vi "CP for Time Vi_MS.vi"(8 "CP A Tag":string[](array[string]), 11 "CP Profile Table for All Seql":string[][](table)) -> (3 "CPIDXZ":T1)   [LabVIEW 2018]
panel:
  out "M_MxRight_No":string[](array[string])
  out "M_RRead_Seq":string[](array[string])
  out "Mx Right No":string[](array[string])
  out "Mx Right Read Seq":string[](array[string])
  out "Assinged Sequence":string[](array[string])
  out "Direction":string[](array[string])
  out "MS_IDX":string[](array[string])
  out "Mx Intensity level [pA]":string[](array[string])
  out "BLX Level [pA]":string[](array[string])
  out "Signal Intensity [pA]":string[](array[string])
  out "S/N ratio":string[](array[string])
  out "S#_IDX":string[](array[string])
  out "L#_IDX":string[](array[string])
  out "AS IDX":string[](array[string])
  out "CP T IDX End [n]":string[](array[string])
  out "CP T IDX Start [n]":string[](array[string])
  out "サイズ":i32
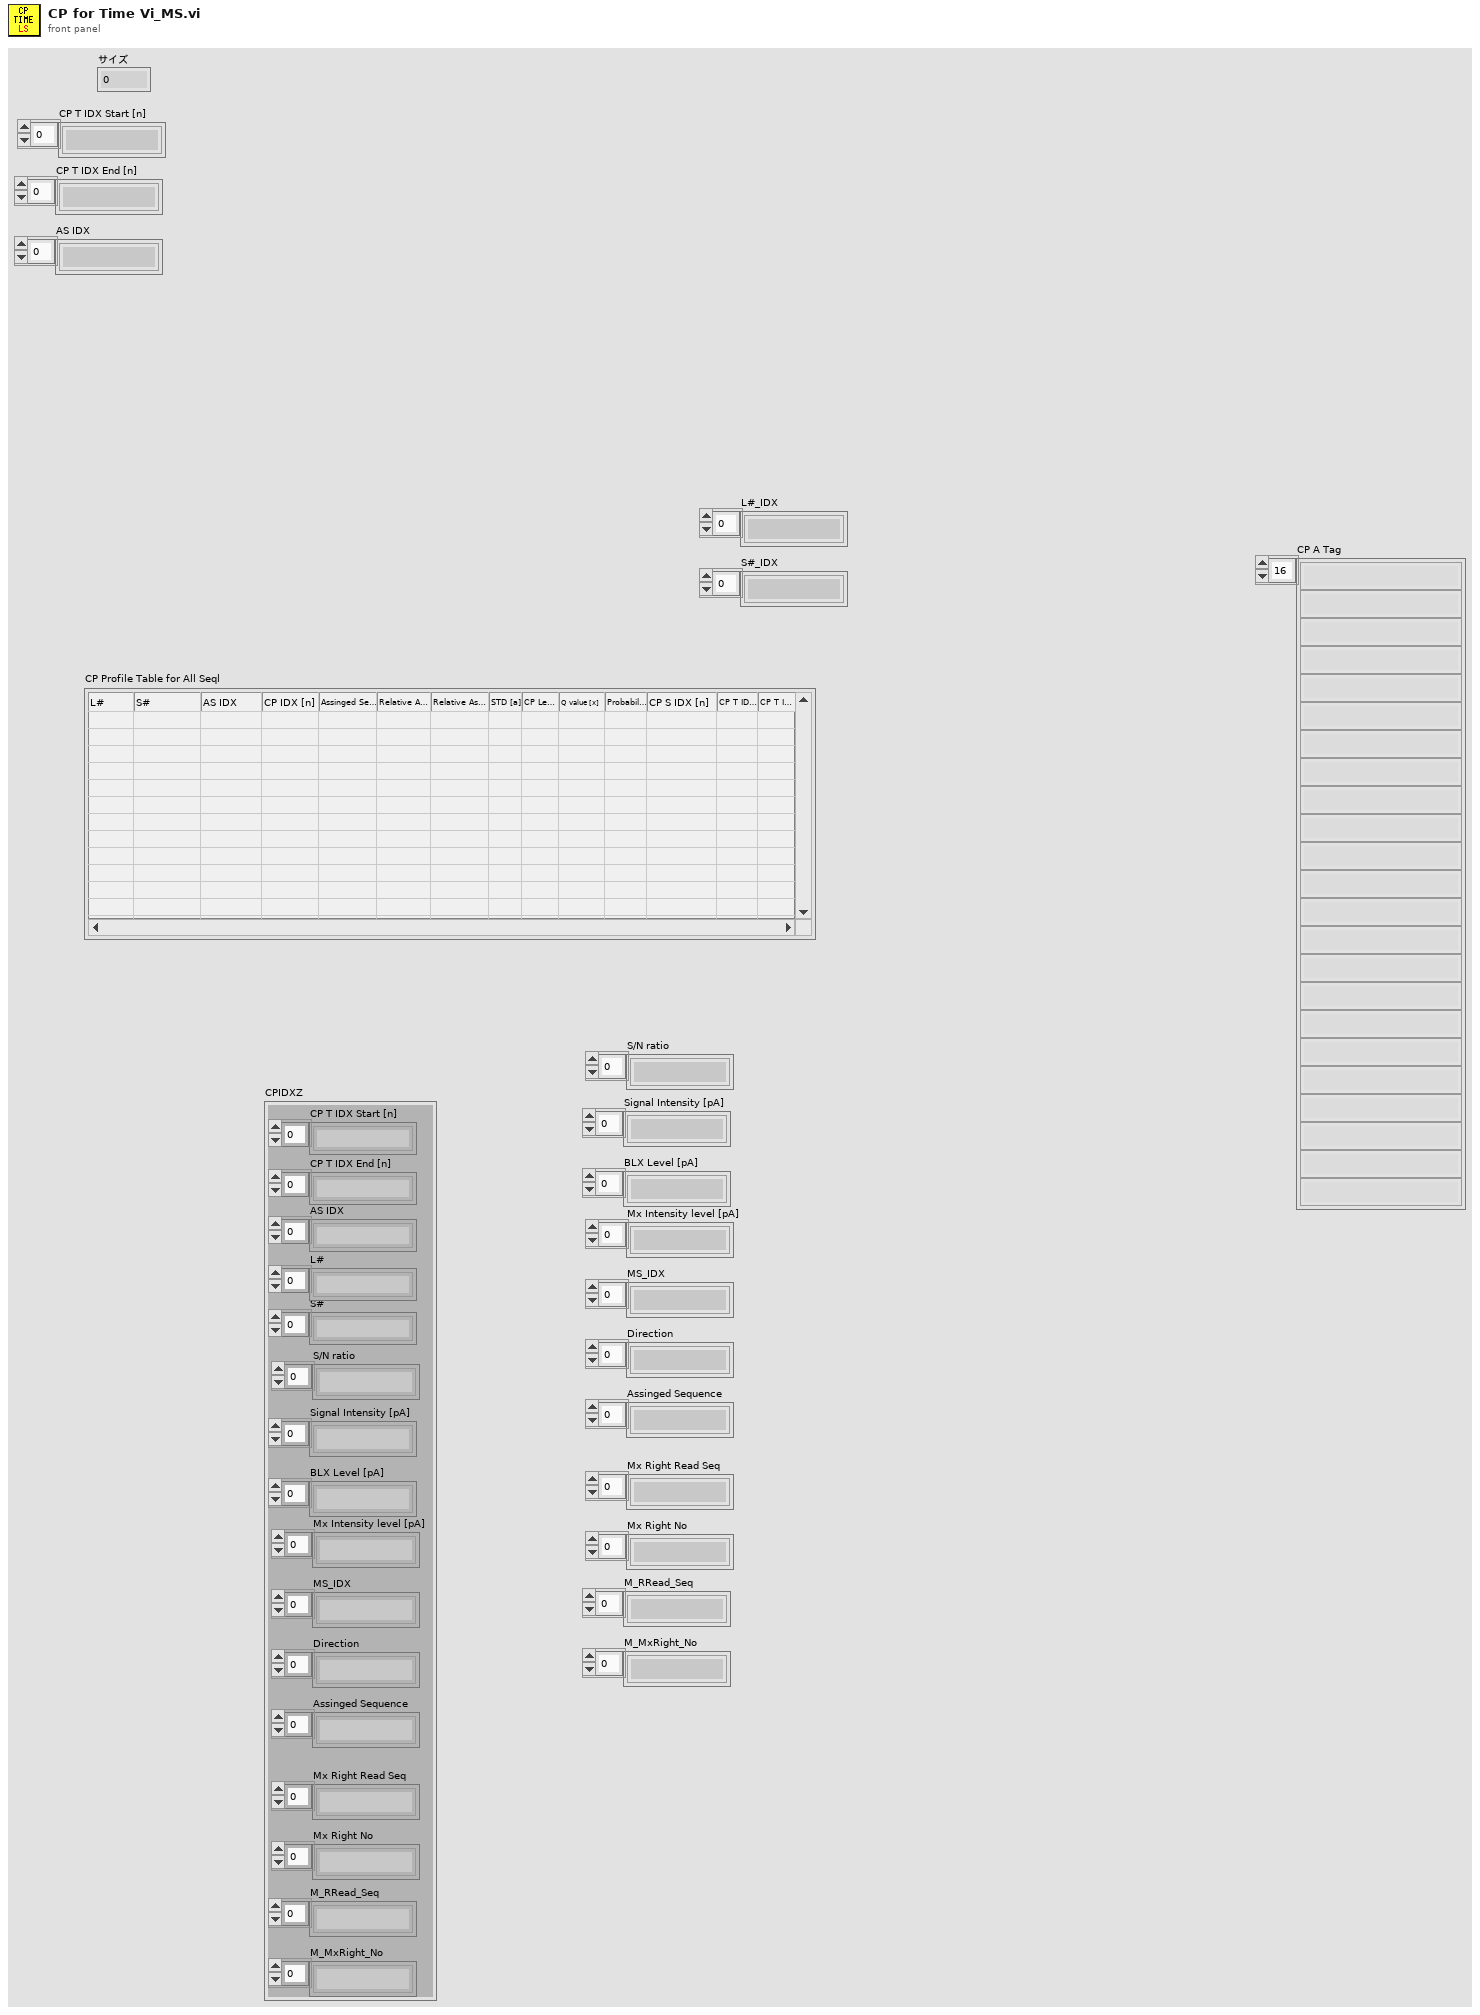
[diagram p1: front panel]
types:
  T1 = cluster{"CP T IDX Start [n]":string[], "CP T IDX End [n]":string[], "AS IDX":string[], "L#":string[], "S#":string[], "S/N ratio":string[], "Signal Intensity [pA]":string[], "BLX Level [pA]":string[], "Mx Intensity level [pA]":string[], "MS_IDX":string[], "Direction":string[], "Assinged Sequence":string[], "Mx Right Read Seq":string[], "Mx Right No":string[], "M_RRead_Seq":string[], "M_MxRight_No":string[]}
  T2 = cluster{string[], string[], string[], string[], string[], string[], string[], string[], string[], string[], string[], string[], string[], string[], string[], string[]}
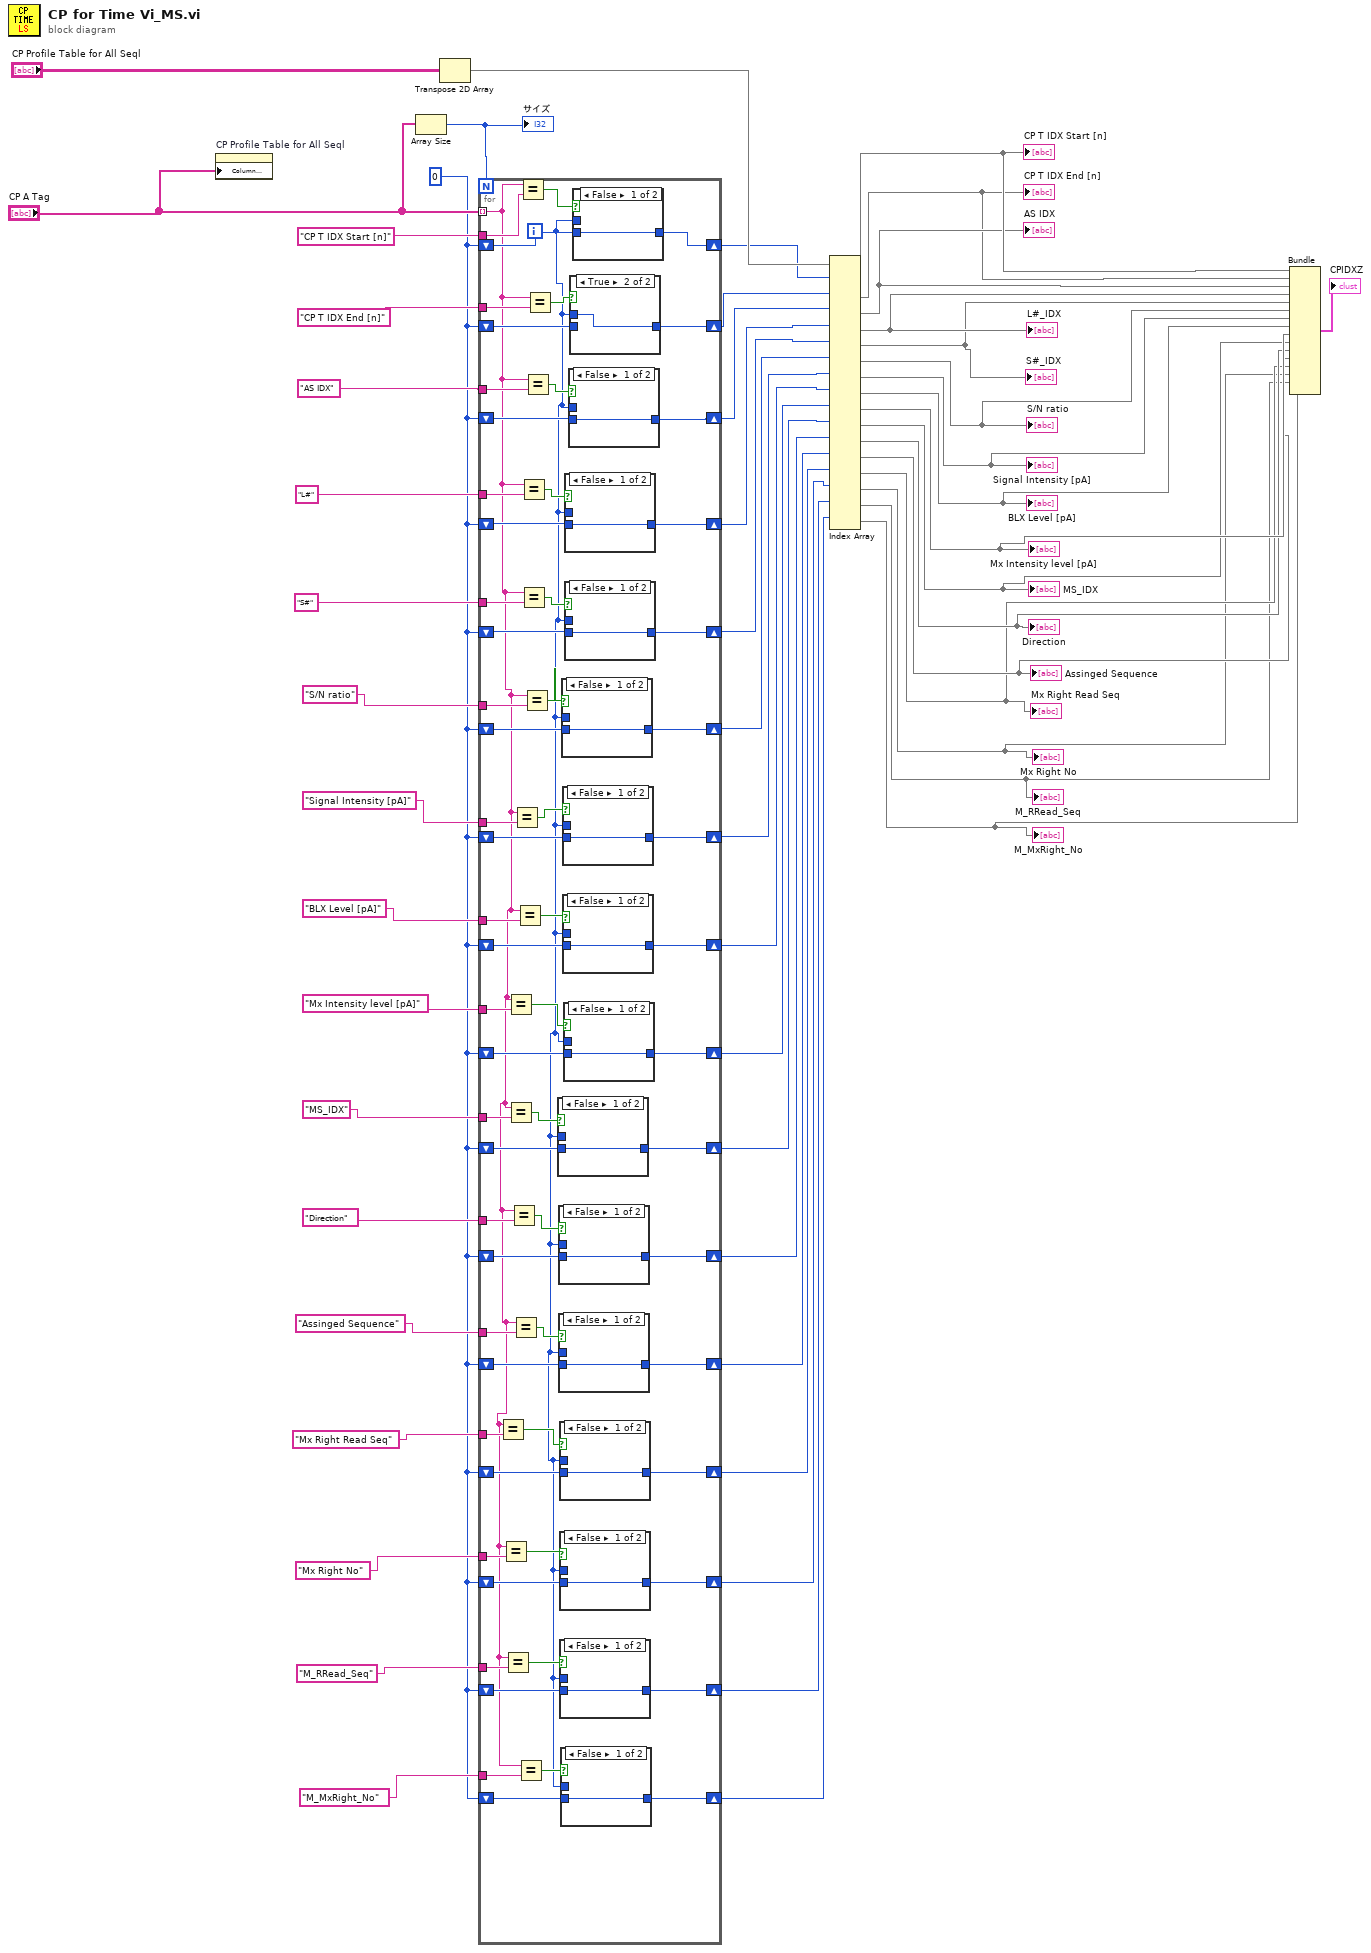
[diagram p0: block diagram]
diagram:
  w24 = 0
  n1 = property on="CP Profile Table for All Seql" class="Tbl (strict)"("Column Headers[]"="CP A Tag") -> ()  [unwired: 2 in, 2 out]
  n2 = Array Size(array="CP A Tag") -> (size(s)=w54:i32)
  "サイズ" <- w54
  n3 = Transpose 2D Array(2D array="CP Profile Table for All Seql") -> (transposed array=w53:string[][])
  n4 = for {
    N: w54 -> [_]
    tunnel: "CP A Tag" -> [w61] mode=indexing
    tunnel: "CP T IDX Start [n]" -> [w120]
    shift-right: [w118] -> w51
    shift-left: w24 -> [w119]
    shift-right: [w115] -> w50
    shift-left: w24 -> [w116]
    shift-right: [w113] -> w49
    shift-left: w24 -> [w114]
    tunnel: "CP T IDX End [n]" -> [w111]
    tunnel: "AS IDX" -> [w110]
    tunnel: "L#" -> [w106]
    tunnel: "S#" -> [w105]
    shift-right: [w104] -> w42
    shift-left: w24 -> [w101]
    shift-right: [w103] -> w41
    shift-left: w24 -> [w102]
    tunnel: "S/N ratio" -> [w100]
    shift-right: [w98] -> w23
    shift-left: w24 -> [w97]
    tunnel: "Signal Intensity [pA]" -> [w95]
    shift-right: [w94] -> w22
    shift-left: w24 -> [w93]
    shift-right: [w91] -> w21
    shift-left: w24 -> [w90]
    tunnel: "BLX Level [pA]" -> [w89]
    tunnel: "Mx Intensity level [pA]" -> [w87]
    shift-right: [w86] -> w20
    shift-left: w24 -> [w85]
    tunnel: "MS_IDX" -> [w83]
    shift-right: [w82] -> w19
    shift-left: w24 -> [w81]
    tunnel: "Direction" -> [w79]
    shift-right: [w78] -> w18
    shift-left: w24 -> [w77]
    shift-right: [w76] -> w16
    shift-left: w24 -> [w75]
    tunnel: "Assinged Sequence" -> [w74]
    tunnel: "Mx Right Read Seq" -> [w72]
    shift-right: [w70] -> w15
    shift-left: w24 -> [w69]
    tunnel: "Mx Right No" -> [w67]
    shift-right: [w66] -> w14
    shift-left: w24 -> [w65]
    tunnel: "M_RRead_Seq" -> [w64]
    shift-right: [w63] -> w13
    shift-left: w24 -> [w62]
    tunnel: "M_MxRight_No" -> [w60]
    shift-right: [w56] -> w12
    shift-left: w24 -> [w55]
    i -> [w57]
    n5 = Equal?(x=w61, y=w72) -> (x = y?=w71:bool)
    n6 = Equal?(x=w61, y=w67) -> (x = y?=w68:bool)
    n7 = Equal?(x=w61, y=w64) -> (x = y?=w58:bool)
    n8 = Equal?(x=w61, y=w87) -> (x = y?=w88:bool)
    n9 = Equal?(x=w61, y=w83) -> (x = y?=w84:bool)
    n10 = Equal?(x=w61, y=w79) -> (x = y?=w80:bool)
    n11 = Equal?(x=w61, y=w74) -> (x = y?=w73:bool)
    n12 = Equal?(x=w61, y=w95) -> (x = y?=w96:bool)
    n13 = Equal?(x=w61, y=w89) -> (x = y?=w92:bool)
    n14 = Equal?(x=w61, y=w60) -> (x = y?=w59:bool)
    n15 = Equal?(x=w61, y=w120) -> (x = y?=w117:bool)
    n16 = Equal?(x=w61, y=w106) -> (x = y?=w108:bool)
    n17 = Equal?(x=w61, y=w105) -> (x = y?=w107:bool)
    n18 = Equal?(x=w61, y=w100) -> (x = y?=w99:bool)
    n19 = Equal?(x=w61, y=w110) -> (x = y?=w109:bool)
    n20 = Equal?(x=w61, y=w111) -> (x = y?=w112:bool)
    n21 = case shown="False" w84 {
      tunnel: w57 -> [_ w134]
      tunnel: [w133 w134] -> w82
      tunnel: w81 -> [w133 _]
      frame False {
      }
      frame True {
      }
    }
    n22 = case shown="False" w80 {
      tunnel: w57 -> [_ w132]
      tunnel: [w131 w132] -> w78
      tunnel: w77 -> [w131 _]
      frame False {
      }
      frame True {
      }
    }
    n23 = case shown="False" w73 {
      tunnel: w57 -> [_ w130]
      tunnel: [w129 w130] -> w76
      tunnel: w75 -> [w129 _]
      frame False {
      }
      frame True {
      }
    }
    n24 = case shown="False" w71 {
      tunnel: w57 -> [_ w128]
      tunnel: [w127 w128] -> w70
      tunnel: w69 -> [w127 _]
      frame False {
      }
      frame True {
      }
    }
    n25 = case shown="False" w68 {
      tunnel: w57 -> [_ w126]
      tunnel: [w125 w126] -> w66
      tunnel: w65 -> [w125 _]
      frame False {
      }
      frame True {
      }
    }
    n26 = case shown="False" w58 {
      tunnel: w57 -> [_ w124]
      tunnel: [w123 w124] -> w63
      tunnel: w62 -> [w123 _]
      frame False {
      }
      frame True {
      }
    }
    n27 = case shown="False" w59 {
      tunnel: w57 -> [_ w122]
      tunnel: [w121 w122] -> w56
      tunnel: w55 -> [w121 _]
      frame False {
      }
      frame True {
      }
    }
    n28 = case shown="False" w99 {
      tunnel: w57 -> [_ w142]
      tunnel: [w141 w142] -> w98
      tunnel: w97 -> [w141 _]
      frame False {
      }
      frame True {
      }
    }
    n29 = case shown="False" w96 {
      tunnel: w57 -> [_ w140]
      tunnel: [w139 w140] -> w94
      tunnel: w93 -> [w139 _]
      frame False {
      }
      frame True {
      }
    }
    n30 = case shown="False" w92 {
      tunnel: w57 -> [_ w138]
      tunnel: [w137 w138] -> w91
      tunnel: w90 -> [w137 _]
      frame False {
      }
      frame True {
      }
    }
    n31 = case shown="False" w88 {
      tunnel: w57 -> [_ w136]
      tunnel: [w135 w136] -> w86
      tunnel: w85 -> [w135 _]
      frame False {
      }
      frame True {
      }
    }
    n32 = case shown="False" w108 {
      tunnel: w57 -> [_ w146]
      tunnel: [w145 w146] -> w104
      tunnel: w101 -> [w145 _]
      frame False {
      }
      frame True {
      }
    }
    n33 = case shown="False" w107 {
      tunnel: w57 -> [_ w144]
      tunnel: [w143 w144] -> w103
      tunnel: w102 -> [w143 _]
      frame False {
      }
      frame True {
      }
    }
    n34 = case shown="False" w109 {
      tunnel: w57 -> [_ w148]
      tunnel: [w147 w148] -> w113
      tunnel: w114 -> [w147 _]
      frame False {
      }
      frame True {
      }
    }
    n35 = case shown="True" w112 {
      tunnel: w57 -> [_ w150]
      tunnel: [w149 w150] -> w115
      tunnel: w116 -> [w149 _]
      frame False {
      }
      frame True {
      }
    }
    n36 = case shown="False" w117 {
      tunnel: w57 -> [_ w152]
      tunnel: [w151 w152] -> w118
      tunnel: w119 -> [w151 _]
      frame False {
      }
      frame True {
      }
    }
  }
  n37 = Index Array(array=w53, index (row) #1=w51, index (row) #2=w50, index (row) #3=w49, index (row) #4=w42, index (row) #5=w41, index (row) #6=w23, index (row) #7=w22, index (row) #8=w21, index (row) #9=w20, index (row) #10=w19, index (row) #11=w18, index (row) #12=w16, index (row) #13=w15, index (row) #14=w14, index (row) #15=w13, index (row) #16=w12) -> (element #1=w40:string[], element #2=w17:string[], element #3=w39:string[], element #4=w38:string[], element #5=w37:string[], element #6=w11:string[], element #7=w10:string[], element #8=w9:string[], element #9=w8:string[], element #10=w7:string[], element #11=w6:string[], element #12=w5:string[], element #13=w4:string[], element #14=w3:string[], element #15=w2:string[], element #16=w1:string[])  [unwired: 16 in]
  "CP T IDX Start [n]" <- w40
  "CP T IDX End [n]" <- w17
  "AS IDX" <- w39
  "L#_IDX" <- w38
  "S#_IDX" <- w37
  "S/N ratio" <- w11
  "Signal Intensity [pA]" <- w10
  "BLX Level [pA]" <- w9
  "Mx Intensity level [pA]" <- w8
  "MS_IDX" <- w7
  "Direction" <- w6
  "Assinged Sequence" <- w5
  "Mx Right Read Seq" <- w4
  "Mx Right No" <- w3
  "M_RRead_Seq" <- w2
  "M_MxRight_No" <- w1
  n38 = Bundle(w40, w17, w39, w38, w37, w11, w10, w9, w8, w7, w6, w5, w4, w3, w2, w1) -> (→"CPIDXZ":T2)  [unwired: 1 in]
